vi "Get Generic Slave Data.vi"(8 "error in (no error)":errorcluster caption="Fehler (Eingang, kein Fehler)", 11 "EtherCAT Slave In":T9 {"VS ref" format="%.0x"}) -> (0 "error out":errorcluster caption="Fehler (Ausgang)", 3 "EtherCAT Slave out":T1 {"I/O Output Data"."BD Refs"."Data Reference" format="%.0x"; "I/O Input Data"."BD Refs"."Data Reference" format="%.0x"; "I/O Output Vars"."VS ref" format="%.0x"; "I/O Imput Vars"."VS ref" format="%.0x"; "VS ref" format="%.0x"})   [LabVIEW 2027, in "SEECD Engine.lvlib"]
uses:
  SEECD Engine.lvlib
  <vilib>/NI VeriStand/Custom Device API/Custom Device Item Ref.ctl
  Type Defs/Generic ECAT Slave Data Cluster.ctl
  Type Defs/Generic ECAT Slave IOV Cluster.ctl
  Shared/Type Defs/UDV Data Type.ctl
  Type Defs/Input Data.ctl
  <vilib>/NI VeriStand/Custom Device API/Block Data Reference.ctl
  <vilib>/NI VeriStand/Custom Device API/Data Reference.ctl
  Type Defs/Output Data.ctl
  Shared/Globals/Property Strings.vi
  <vilib>/NI VeriStand/Custom Device API/Get Item Property (Boolean).vi
  Shared/SEECD Shared.lvlib
  <vilib>/NI VeriStand/Custom Device API/Custom Device API.lvlib
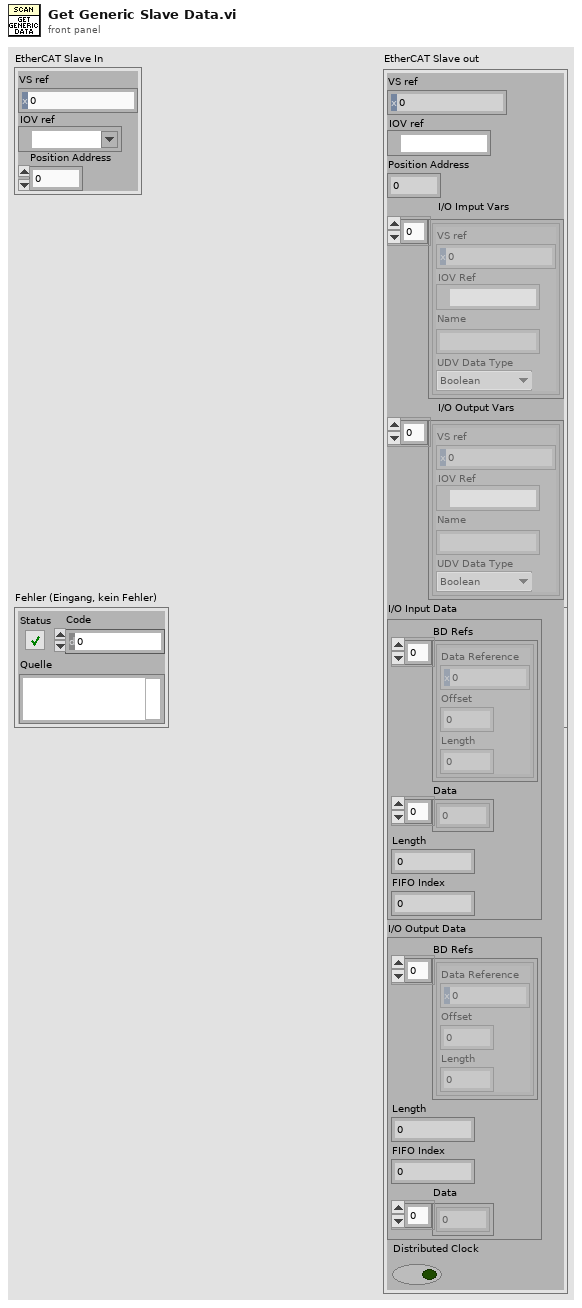
[diagram p1: front panel]
types:
  T1 = typedef "SEECD Engine.lvlib/Generic ECAT Slave Data Cluster.ctl" = cluster{"VS ref":T2, "IOV ref":refnum<k21>, "Position Address":u16, "I/O Imput Vars ":T3[], "I/O Output Vars":T3[], "I/O Input Data":T5, "I/O Output Data":T8, "Distributed Clock":bool}
  T2 = typedef "Custom Device API.lvlib/Custom Device Item Ref.ctl" = u64
  T3 = typedef "SEECD Engine.lvlib/Generic ECAT Slave IOV Cluster.ctl" = cluster{"VS ref":T2, "IOV Ref":refnum<k21>, "Name":string, "UDV Data Type":T4}
  T4 = typedef "SEECD Shared.lvlib/UDV Data Type.ctl" = enum16{"Boolean", "Fixed Point", "Int8", "Int16", "Int32", "Int64", "U32 Bit Field", "UInt8", "UInt16", "UInt32", "UInt64", "Other", "DBL", "SGL"}
  T5 = typedef "SEECD Engine.lvlib/Input Data.ctl" = cluster{"BD Refs":T6[], "Data":dbl[], "Length":i32, "FIFO Index":i32}
  T6 = typedef "Custom Device API.lvlib/Block Data Reference.ctl" = cluster{"Data Reference":T7, "Offset":u64, "Length":u64}
  T7 = typedef "Custom Device API.lvlib/Data Reference.ctl" = i32
  T8 = typedef "SEECD Engine.lvlib/Output Data.ctl" = cluster{"BD Refs":T6[], "Length":i32, "FIFO Index":i32, "Data":dbl[]}
  T9 = cluster{"VS ref":T2, "IOV ref":refnum<k21>, "Position Address":u16}
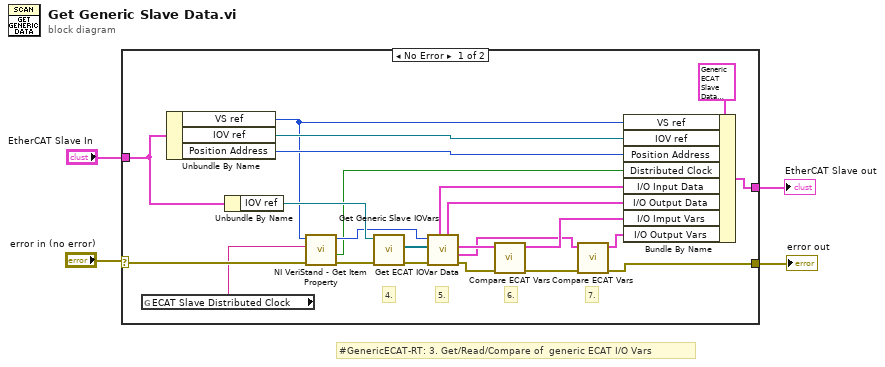
[diagram p0: block diagram]
diagram:
  # "#GenericECAT-RT: 3. Get/Read/Compare of  generic ECAT I/O Vars"
  n1 = case shown="No Error" "error in (no error)" {
    selector: "error in (no error)" -> [w9 w28]
    tunnel: "EtherCAT Slave In" -> [w26 _]
    tunnel: [w18 w28] -> w2
    tunnel: [w25 _] -> w1
    frame No Error {
      # "7."
      # "6."
      # "5."
      # "4."
      n2 = global read "Property Strings.vi" "ECAT Slave Distributed Clock"() -> (w6:string)
      n3 = Unbundle By Name(w26) -> ("VS ref"=w8:T2, "IOV ref"=w11:refnum<k21>, "Position Address"=w21:u16)
      n4 = Unbundle By Name(w26) -> ("IOV ref"=w23:refnum<k21>)
      n5 = call-poly <vilib>:"NI VeriStand - Get Item Property.vi"("error in (no error)"=w9, "Property Name"=w6, "Item Ref in"=w8) -> ("error out"=w10:errorcluster, "Value"=w5:bool, "Item Ref out"=w7:T2)  [unwired: 5 in, 1 out]
      n6 = call "Get Generic Slave IOVars.vi"("error in (no error)"=w10, "ECAT Slave in"=w23) -> ("error IO"=w24:errorcluster, "ECAT Variablenobjekt"=w22:refnum<k21>[])  [unwired: 7 in, 1 out]
      n7 = call "Get ECAT IOVar Data.vi"("Fehler (Eingang, kein Fehler)"=w24, "ECAT Variablenobjekt"=w22, "VS ref"=w7) -> ("Fehler (Ausgang)"=w20:errorcluster, "I/O Output Vars"=w12:T3[], "I/O Imput Vars"=w15:T3[], "I/O Output Data"=w16:T8, "I/O Input Data"=w17:T5)  [unwired: 3 in, 1 out]
      n8 = call "Compare ECAT Vars.vi"("Fehler (Eingang, kein Fehler)"=w20, "I/O Output Vars (Eingang)"=w15) -> ("Fehler (Ausgang)"=w19:errorcluster, "I/O Output Vars (Ausgang)"=w14:T3[])  [unwired: 8 in]
      n9 = call "Compare ECAT Vars.vi"("Fehler (Eingang, kein Fehler)"=w19, "I/O Output Vars (Eingang)"=w12) -> ("Fehler (Ausgang)"=w18:errorcluster, "I/O Output Vars (Ausgang)"=w13:T3[])  [unwired: 8 in]
      n10 = Bundle By Name(cluster=T1 {"VS ref"=0, "IOV ref"="", "Position Address"=0, "I/O Imput Vars "=[], "I/O Output Vars"=[], "I/O Input Data"={"BD Refs"=[], "Data"=[], "Length"=0, "FIFO Index"=0}, "I/O Output Data"={"BD Refs"=[], "Length"=0, "FIFO Index"=0, "Data"=[]}, "Distributed Clock"=FALSE} ("EtherCAT Slave"), "VS ref"=w8, "IOV ref"=w11, "Position Address"=w21, "Distributed Clock"=w5, "I/O Input Data"=w17, "I/O Output Data"=w16, "I/O Imput Vars"=w14, "I/O Output Vars"=w13) -> (w25:T1)
    }
    frame Error {
    }
  }
  "error out" <- w2
  "EtherCAT Slave out" <- w1
